vi "VHistFile - Application directory path.vi"() -> (0 "application directory path":path)   [LabVIEW 2021]
doc: "The VI returns a directory path of the top-level VI in a chain of its callers. The returned path includes neither a VI library name nor an executable file name if the top-level VI resides within either of them. The VI always returns a directory path.\n\n::: CalcExpress Toolkit :::\nCopyright (c) 2000-2026 Konstantin Shifershteyn. All rights reserved."
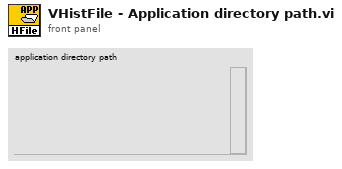
[diagram p1: front panel]
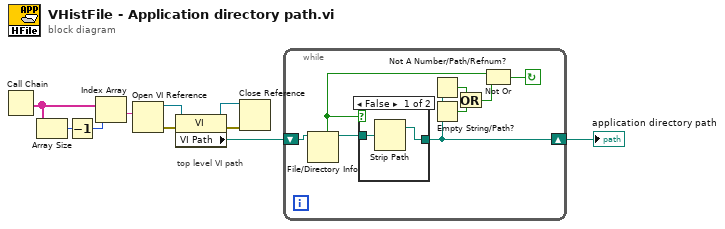
[diagram p0: block diagram]
diagram:
  # "top level VI path"
  n1 = Call Chain() -> (call chain=w3:string[])
  n2 = Array Size(array=w3) -> (size(s)=w4:i32)
  n3 = Decrement(x=w4) -> (x-1=w5:i32)
  n4 = Index Array(array=w3, index=w5) -> (element=w6:string)
  n5 = Open VI Reference(vi path=w6) -> (vi reference=w7:refnum<vi>, error out=w8:errorcluster)  [unwired: 5 in]
  n6 = property class="VI"(reference=w7, error in=w8) -> (reference out=w10:refnum<vi>, error out=w9:errorcluster, "VI Path"=w2:path)
  n7 = Close Reference(reference=w10, error in (no error)=w9) -> ()  [unwired: 1 out]
  n8 = while {
    shift-right: [w16] -> w1
    shift-left: w2 -> [w18]
    stop <- w13 continue-if-true
    n9 = File/Directory Info(path=w18) -> (path out=w17:path, directory=w12:bool)  [unwired: 1 in, 5 out]
    n10 = case shown="False" w12 {
      tunnel: w17 -> [w20 w21]
      tunnel: [w19 w21] -> w16
      frame False {
        n11 = Strip Path(path=w20) -> (stripped path=w19:path)  [unwired: 1 out]
      }
      frame True {
      }
    }
    n12 = Not A Number/Path/Refnum?(number/path/refnum=w16) -> (NaN/Path/Refnum?=w14:bool)
    n13 = Empty String/Path?(string/path=w16) -> (empty?=w15:bool)
    n14 = Or(x=w14, y=w15) -> (x .or. y?=w11:bool)
    n15 = Not Or(1:w11, 2:w12) -> (0:w13:bool)
  }
  "application directory path" <- w1
